vi "VIH HelpGen - Write HTML File - Poly VI - VI Instance Description.vi"(5 "Save params":T1, 6 "Table Templates":T2, 7 "InstanceRef":string, 8 "error in":errorcluster, 9 "HTML in":string, 10 "VI Path":path, 11 "Project Tree":T3) -> (0 "error out":errorcluster, 1 "HTML out":string, 3 "dup Project Tree":T3)   [LabVIEW 2014]
doc: "::: VI Helpeks :::\nCopyright (c) 2000-2026 Konstantin Shifershteyn. All rights reserved."
uses:
  _VIH Project Manager.llb/VIH Project Tree Typedef - Tree Refnum.ctl
  VIH HelpGen Typedef - Table Templates Cluster - VI Help.ctl
panel:
  # "VI Helpeks\nCopyright (c) 2012-2026 Konstantin Shifershteyn"
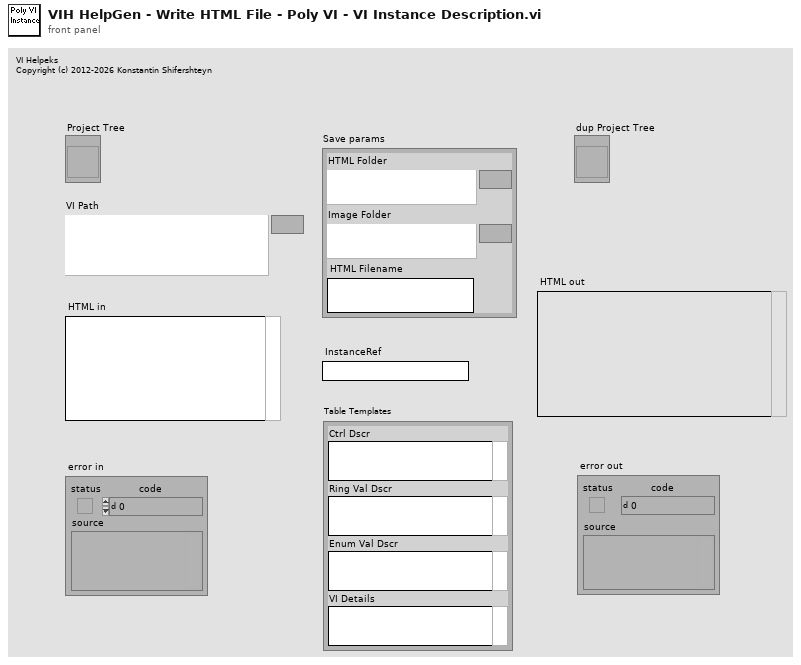
[diagram p1: front panel]
types:
  T1 = cluster{"HTML Folder":path, "Image Folder":path, "HTML Filename":string}
  T2 = typedef "VIH HelpGen Typedef - Table Templates Cluster - VI Help.ctl" = cluster{"Ctrl Dscr":string, "Ring Val Dscr":string, "Enum Val Dscr":string, "VI Details":string}
  T3 = typedef "VIH Project Tree Typedef - Tree Refnum.ctl" = refnum<vi>
  T4 = typedef "VIH HelpGen Typedef - Cluster - File Rule.ctl" = cluster{"OutName":string, "BuildHelp":T5, "Source Paths":T6, "Target Paths":T7, "DscrMode":T8, "Description":string, "Control Rules":T9[], "Flags":T11, "Ctl_DscrMode":T8, "Ctl_ClustMembers":T5, "Ctl_EnumValues":T5, "MenuItemIcons":T5, "%Comments":string, "DetailsMode":T8, "DetailsText":string, "ProductInfoMode":T5, "ProductInfoText":string}
  T5 = typedef "VIH HelpGen Typedef - Enum - Default,Enable,Disable.ctl" = enum16{"Default", "Enable", "Disable"}
  T6 = typedef "VIH HelpGen Typedef - Cluster - File Rule - Source Paths.ctl" = cluster{"CSS Files":path[], "JS Files":path[], "Html Template":path}
  T7 = typedef "VIH HelpGen Typedef - Cluster - File Rule - Target Paths.ctl" = cluster{"HTML Dir":path, "Image Dir":path, "CSS Dir":path, "JS Dir":path}
  T8 = typedef "VIH HelpGen Typedef - Enum - Description Mode.ctl" = enum16{"Default", "Description", "Description1", "Description2", "Custom", "None"}
  T9 = typedef "VIH HelpGen Typedef - Cluster - Control Rule.ctl" = cluster{"CtrlID":string, "CustomRule":bool, "DscrMode":T8, "Description":string, "ClusterMembers":T5, "EnumValues":T5, "EnumValDscr":T10[], "CustomName":string}
  T10 = typedef "VIH HelpGen Typedef - Cluster - Enum Value Info.ctl" = cluster{"Value":ext, "String":string, "Description":string}
  T11 = typedef "VIH HelpGen Typedef - Cluster - Group Rule - Flags.ctl" = cluster{"Override CSS Files":bool, "Override JS Files":bool, "Override Ctl Rules":bool}
  T12 = typedef "imagedata.ctl" = cluster{"image type":i32, "image depth":i32, "image":u8[], "mask":u8[], "colors":u32[], "Rectangle":cluster{"left":i16, "top":i16, "right":i16, "bottom":i16}}
  T13 = cluster{"Original VI Name":string, "Conpane Image":T12}
  T14 = cluster{string[], "Control Rules":T9[], "Ctl_DscrMode":T8, "Ctl_ClustMembers":T5, "Ctl_EnumValues":T5}
  T15 = cluster{"HTML Folder":path, "directory path out":path, "HTML Filename":string}
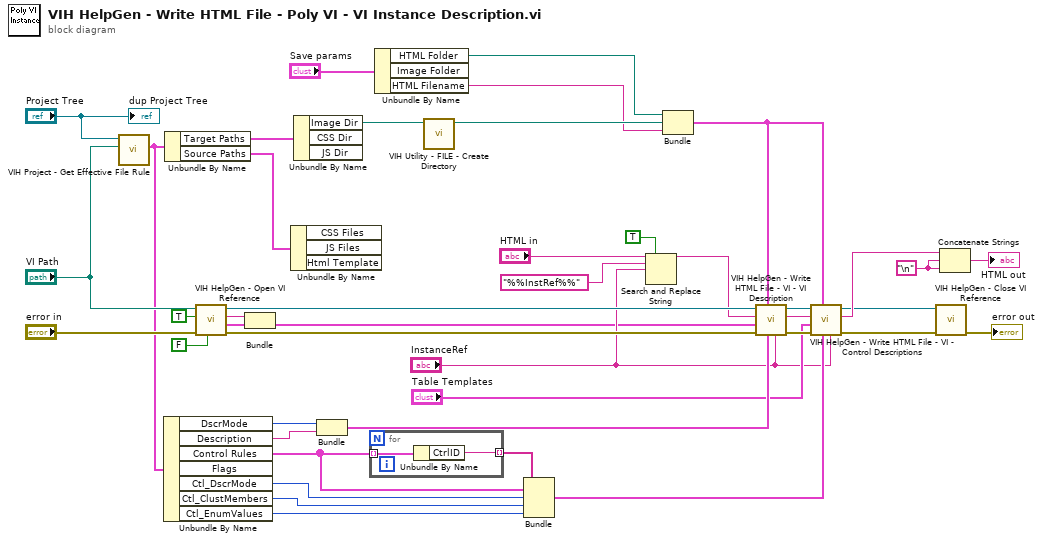
[diagram p0: block diagram]
diagram:
  w11 = "\n"
  n1 = call "VIH Project - Get Effective File Rule.vi"("File Path"="VI Path", "Project Tree"="Project Tree") -> ("Effective File Rule"=w33:T4)  [unwired: 6 in, 3 out]
  n2 = Unbundle By Name(w33) -> ("DscrMode"=w32:T8, "Description"=w31:string, "Control Rules"=w26:T9[], "Ctl_DscrMode"=w29:T8, "Ctl_ClustMembers"=w28:T5, "Ctl_EnumValues"=w27:T5)  [unwired: 1 out]
  n3 = Unbundle By Name(w33) -> ("Target Paths"=w38:T7, "Source Paths"=w37:T6)
  n4 = call "VIH HelpGen - Open VI Reference.vi"("Enable Conpane Image Check (T)"=FALSE, "error in"="error in", "Force use wrapper (F)"=TRUE, "VI Path"="VI Path") -> ("error out"=w19:errorcluster, "Conpane Image"=w9:T12, "Original VI Name"=w23:string, "VI Reference"=w39:refnum<vi>)  [unwired: 4 in]
  n5 = Bundle("Original VI Name"=w23, "Conpane Image"=w9) -> (w10:T13)  [unwired: 1 in]
  n6 = Unbundle By Name(w37) -> ()  [unwired: 3 out]
  n7 = Unbundle By Name(w38) -> ("Image Dir"=w34:path)  [unwired: 2 out]
  n8 = Bundle("DscrMode"=w32, "Description"=w31) -> (w30:cluster{"DscrMode":T8, "Description":string})  [unwired: 1 in]
  n9 = for {
    tunnel: w26 -> [w45] mode=indexing
    tunnel: [w44] -> w25 mode=indexing
    n10 = Unbundle By Name(w45) -> ("CtrlID"=w44:string)
  }
  n11 = Unbundle By Name("Save params") -> ("HTML Folder"=w2:path, "HTML Filename"=w1:string)  [unwired: 1 out]
  n12 = call "VIH Utility - FILE - Create Directory.vi"("directory path"=w34) -> ("directory path out"=w5:path)  [unwired: 6 in, 2 out]
  n13 = Bundle(w25, "Control Rules"=w26, "Ctl_DscrMode"=w29, "Ctl_ClustMembers"=w28, "Ctl_EnumValues"=w27) -> (w24:T14)  [unwired: 1 in]
  n14 = Search and Replace String(replace all?=TRUE, input string="HTML in", search string="%%InstRef%%", replace string="InstanceRef") -> (result string=w14:string)  [unwired: 4 in, 3 out]
  n15 = Bundle("HTML Folder"=w2, "directory path out"=w5, "HTML Filename"=w1) -> (w4:T15)  [unwired: 1 in]
  n16 = call "VIH HelpGen - Write HTML File - VI - VI Description.vi"("InstanceRef"="InstanceRef", "Description Params"=w30, "Save params"=w4, "error in"=w19, "Original VI Info"=w10, "HTML in"=w14, "VI Reference"=w39) -> ("error out"=w41:errorcluster, "HTML out"=w40:string, "dup VI Reference"=w42:refnum<vi>)  [unwired: 2 in]
  n17 = call "VIH HelpGen - Write HTML File - VI - Control Descriptions.vi"("InstanceRef"="InstanceRef", "Ctrl Dscr Params"=w24, "Save params"=w4, "error in"=w41, "Table Templates"="Table Templates", "HTML in"=w40, "VI Reference"=w42) -> ("error out"=w8:errorcluster, "HTML out"=w13:string, "dup VI Reference"=w7:refnum<vi>)  [unwired: 2 in]
  n18 = call "VIH HelpGen - Close VI Reference.vi"("error in"=w8, "VI Reference"=w7) -> ("error out"=→"error out":errorcluster)  [unwired: 9 in]
  n19 = Concatenate Strings(w13, w11, w11) -> (→"HTML out":string)
  "dup Project Tree" <- "Project Tree"
